vi "example sequence single sample gen.vi"(10 "frequency":dbl=100.0 format="%0.2f", 11 "amplitude":dbl=1.0 format="%0.2f") -> (2 "sine wave":dbl format="%0.2f", 3 "timestamp":timestamp)   [LabVIEW 2020]
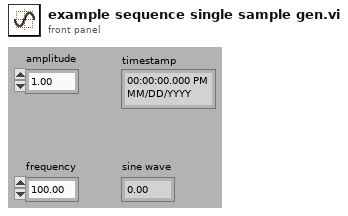
[diagram p1: front panel]
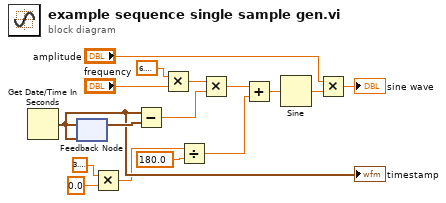
[diagram p0: block diagram]
diagram:
  n1 = Get Date/Time In Seconds() -> (seconds since 1Jan1904=w15:timestamp)
  "timestamp" <- w15
  n2 = feedback-in #1(w15) -> ()
  n3 = feedback #1(w15) -> (w16:timestamp)
  n4 = Multiply(x=3.141592653589793, y=0.0 ("phase")) -> (x*y=w4:dbl)
  n5 = Subtract(x=w15, y=w16) -> (x-y=w14:dbl)
  n6 = Multiply(x=6.283185307179586, y="frequency") -> (x*y=w2:dbl)
  n7 = Divide(x=w4, y=180.0) -> (x/y=w9:dbl)
  n8 = Multiply(x=w2, y=w14) -> (x*y=w8:dbl)
  n9 = Add(x=w8, y=w9) -> (x+y=w6:dbl)
  n10 = Sine(x=w6) -> (sin(x)=w7:dbl)
  n11 = Multiply(x="amplitude", y=w7) -> (x*y=→"sine wave":dbl)
